vi "Burst.vi"(0 "RFFE Command in":refnum<class "RFFE Command.lvclass">, 1 "Bus Number":i32, 5 "instrument handle in":refnum<k15>, 11 "error in (no error)":errorcluster) -> (4 "RFFE Command out":refnum<class "RFFE Command.lvclass">, 6 "instrument handle out":refnum<k15>, 15 "error out":errorcluster)   [LabVIEW 2018, in "MIPI RFFE API.lvlib" / "RFFE Command.lvclass"]
uses:
  RFFE Command.lvclass
  <instrlib>/niDigital/niDigital.llb/niDigital Burst Pattern (Burst Only).vi
  MIPI RFFE API.lvlib
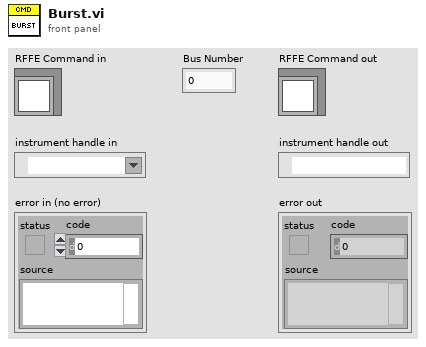
[diagram p1: front panel]
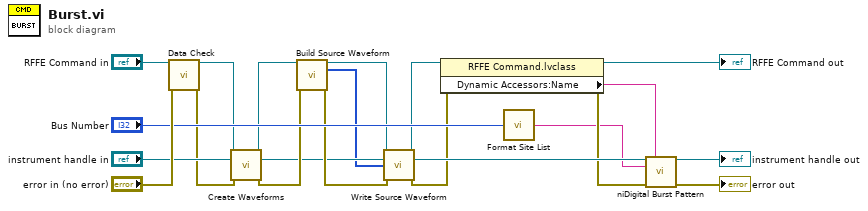
[diagram p0: block diagram]
diagram:
  n1 = call-dynamic "Data Check.vi"("RFFE Command in"="RFFE Command in", "error in (no error)"="error in (no error)") -> ("RFFE Command out"=w14:refnum<class "RFFE Command.lvclass">, "error out"=w12:errorcluster)  [unwired: 12 in]
  n2 = call-dynamic "Create Waveforms.vi"("RFFE Command in"=w14, "instrument handle in"="instrument handle in", "error in (no error)"=w12) -> ("RFFE Command out"=w13:refnum<class "RFFE Command.lvclass">, "instrument handle out"=w6:refnum<k15>, "error out"=w11:errorcluster)  [unwired: 10 in]
  n3 = call-dynamic "Build Source Waveform.vi"("RFFE Command in"=w13, "error in (no error)"=w11) -> ("RFFE Command out"=w9:refnum<class "RFFE Command.lvclass">, "Source Waveform"=w4:u32[], "error out"=w7:errorcluster)  [unwired: 11 in]
  n4 = call-dynamic "Write Source Waveform.vi"("RFFE Command in"=w9, "instrument handle"=w6, "Waveform Data"=w4, "error in (no error)"=w7) -> ("RFFE Command out"=w8:refnum<class "RFFE Command.lvclass">, "instrument handle out"=w5:refnum<k15>, "error out"=w3:errorcluster)  [unwired: 9 in]
  n5 = property class="RFFE Command.lvclass"(reference=w8, error in=w3) -> (reference out=→"RFFE Command out":refnum<class "RFFE Command.lvclass">, error out=w2:errorcluster, "Dynamic Accessors:Name"=w10:string)
  n6 = call "Format Site List.vi"("Bus Number"="Bus Number") -> ("Site List"=w1:string)  [unwired: 14 in]
  n7 = call-poly <instrlib>:"niDigital Burst Pattern.vi"("instrument handle"=w5, "start label"=w10, "site list"=w1, "error in"=w2) -> ("instrument handle out"=→"instrument handle out":refnum<k15>, "error out"=→"error out":errorcluster)  [unwired: 10 in]
